vi "to_json.vi"(8 "error in":errorcluster, 11 "channelConfig in":refnum<class "channelConfig.lvclass">) -> (0 "error out":errorcluster, 2 "json":string, 3 "channelConfig out":refnum<class "channelConfig.lvclass">, 4 "Not Default":bool)   [LabVIEW 2020, in "nominal types.lvlib" / "channelConfig.lvclass"]
uses:
  channelConfig.lvclass
  channelConfig.lvclass/channelConfig.ctl
  e18f592a-8fe0-4010-91a4-70852b3667c2.vi
  383bacbf-beb0-46d4-b203-dcb6afdce316.vi
  <vilib>/JDP Science/JSONtext/Variant to JSON Text.vi
  <vilib>/JDP Science/JSONtext/LVClass Serializer/JSONtext LVClass Serializer.lvclass
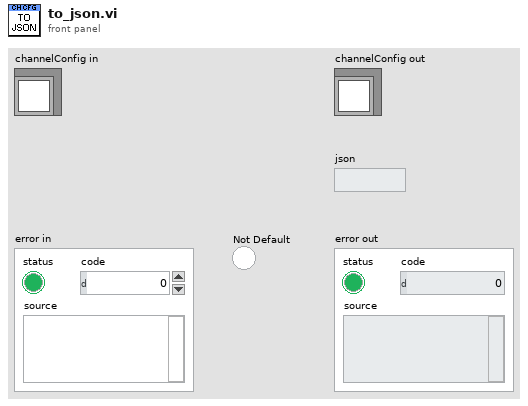
[diagram p1: front panel]
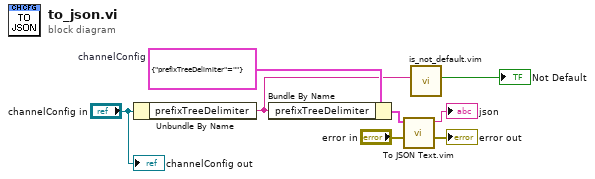
[diagram p0: block diagram]
diagram:
  w7 = cluster{"prefixTreeDelimiter":string} {"prefixTreeDelimiter"=""}  # channelConfig
  n1 = Unbundle By Name("channelConfig in") -> ("prefixTreeDelimiter"=w1:string)
  n2 = Bundle By Name(cluster=w7, "prefixTreeDelimiter"=w1) -> (w3:cluster{"prefixTreeDelimiter":string})
  n3 = call "To JSON Text.vim"("error in (no error)"="error in", "Anything"=w3) -> ("error out"=→"error out":errorcluster, "<JSON>"=→"json":string)  [unwired: 8 in]
  n4 = call "is_not_default.vim"("data"=w1) -> ("Not Default"=→"Not Default":bool)  [unwired: 10 in]
  "channelConfig out" <- "channelConfig in"
